vi "Test-FAMM.vi"() -> ()   [LabVIEW 2020]
doc: "Test the Historian performance"
uses:
  FAMM.lvclass
  HISW/HISW.lvclass
  <vilib>/platform/TimedLoop/XDataNode/XDataNode.xnode
  <vilib>/Platform/TimedLoop/XDataNode/nitl_modes.ctl
  <vilib>/Platform/TimedLoop/XDataNode/XDNodeRunTimeDep.lvlib
  <vilib>/Platform/TimedLoop/XDataNode/wakeup.ctl
  <vilib>/Platform/TimedLoop/XDataNode/timing_clust.ctl
  HISW/controls/typedef_PAQsample.ctl
  DBAL/DBAL.lvclass
  PAQ-memory.lvclass
panel:
  in  "View":bool
  in  "DAQ":bool
  out "# elements in queue":i32
  out "DAQ":picture
  in  "update":bool
  in  "auto":bool
  out "tablename":string
  out "Array":bool[](array[boolean])
  out "PAQpointers":i32[](array[numeric])
  out "XY Graph":cluster{"time":dbl[], "min":dbl[]}[](graph)
  in  "GET_Graph":bool
  in  "Size":i32=1000
  in  "Pointer":i32
  in  "TAG":i32=5 min=0 max=10000
  in  "Layer":i32 min=0
  out "Resolution":dbl format="%#.5p"
  out "Tags":i32
  out "Database configuration":string
  out "37x37":picture
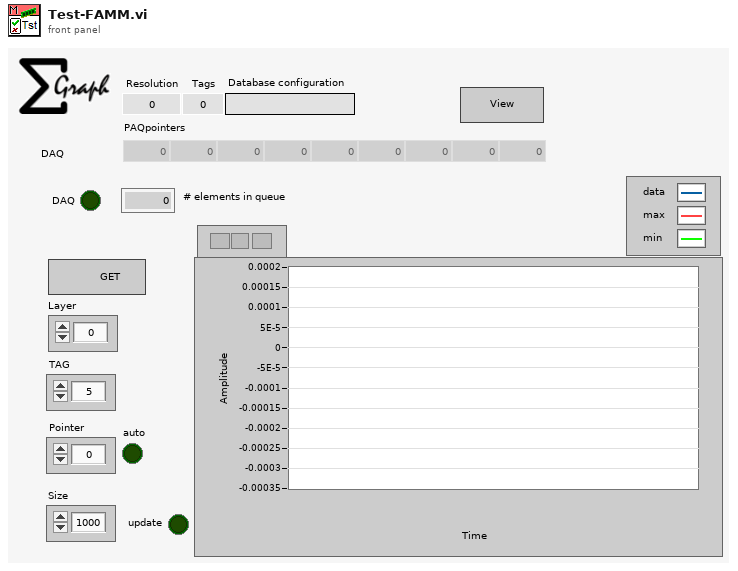
[diagram p1: front panel]
types:
  T1 = typedef "typedef_PAQsample.ctl" = cluster{"Time Stamp":timestamp, "TAGs":string[], "status":u32[], "data":dbl[], "Source":string}
  T2 = typedef "XDNodeRunTimeDep.lvlib/timing_clust.ctl" = cluster{"Expected End [f-1]":u64, "Actual End [f-1]":u64, "Finished Late? [f-1]":bool, "Expected End [i-1]":u64, "Actual End [i-1]":u64, "Finished Late? [i-1]":bool, "Expected Start [i]":u64, "Actual Start [i]":u64, "Expected Start [f]":u64, "Actual Start [f]":u64, "Source Name":string, "Structure Name":string, "Period":i64, "Deadline":i64, "Offset":i64, "Start":i64, "Priority":i32, "Timeout":i32, "Mode":T3, "Wakeup Reason":T4, "Error":errorcluster, "Source Type":string, "Secondary Source Type":string, "Global End Time":u64, "Global Start Time":u64, "Frame Duration":u64, "Iteration Duration":u64, "Assigned CPU":i32, "I/O Scan Engine Mode":u32}
  T3 = typedef "XDNodeRunTimeDep.lvlib/nitl_modes.ctl" = enum32{"No Change", "Process missed periods, maintain original phase", "Discard missed periods, maintain original phase", "Process missed periods, ignore original phase", "Discard missed periods, ignore original phase"}
  T4 = typedef "XDNodeRunTimeDep.lvlib/wakeup.ctl" = enum32{"Normal", "Aborted", "Asynchronous wakeup", "Timing source error", "Timed loop error", "Timeout"}
  T5 = cluster{"TAG":string, "Layer":i32, "Pointer":i32, "Size":i32}
  T6 = cluster{"time":dbl[], "data":dbl[], "max":dbl[], "min":dbl[], "status":u32[]}
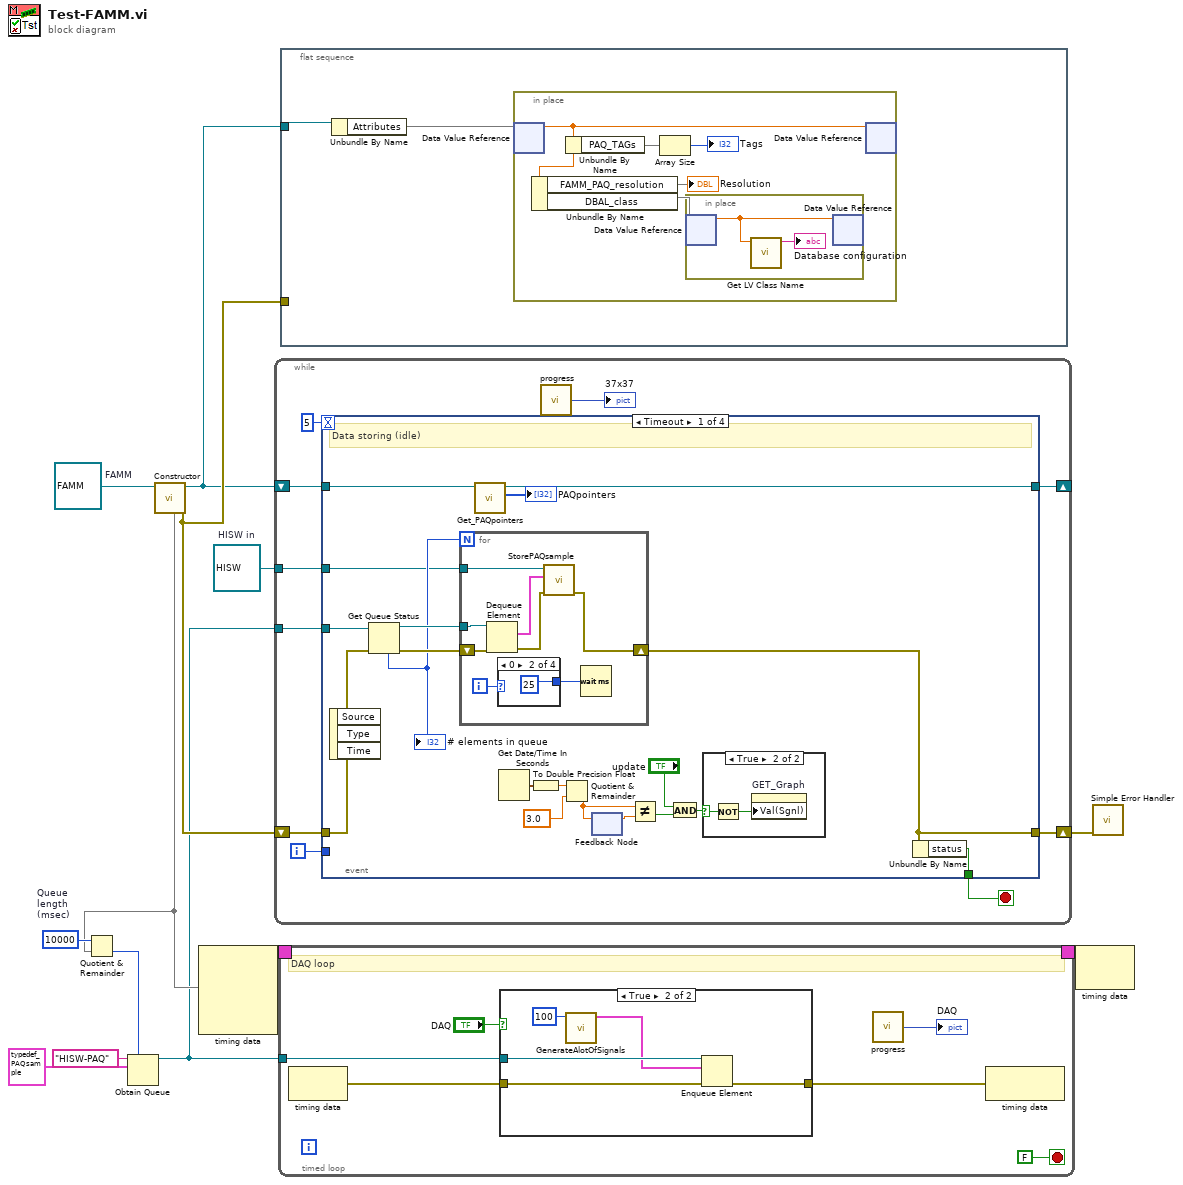
[diagram p0: block diagram]
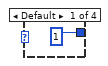
[diagram p3: hidden frame]
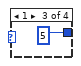
[diagram p4: hidden frame]
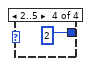
[diagram p5: hidden frame]
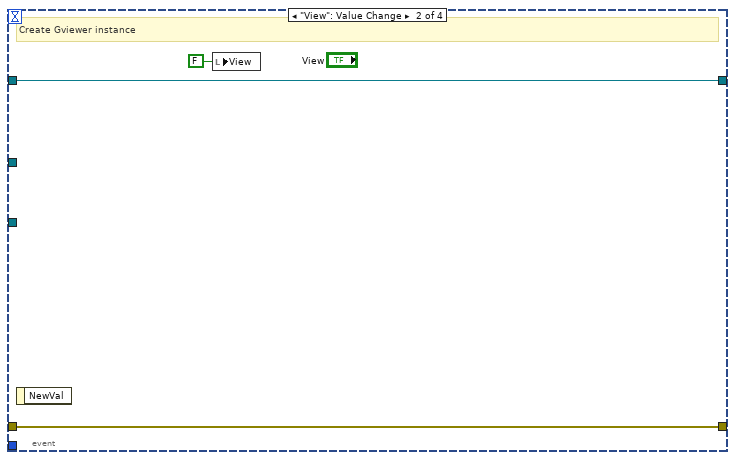
[diagram p7: hidden frame]
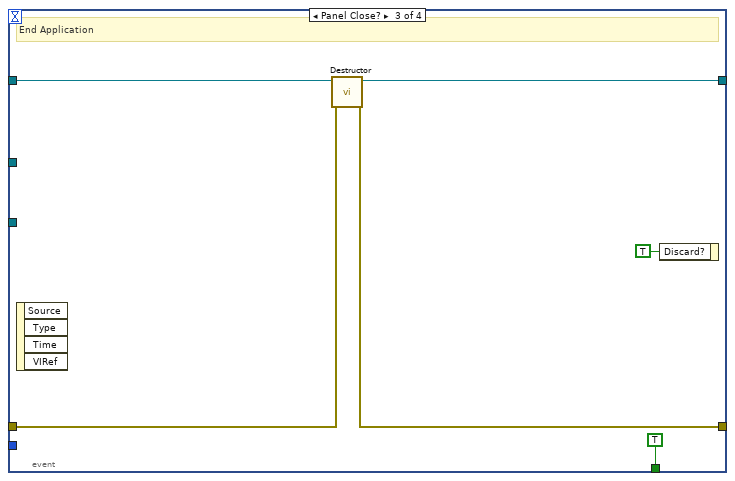
[diagram p8: hidden frame]
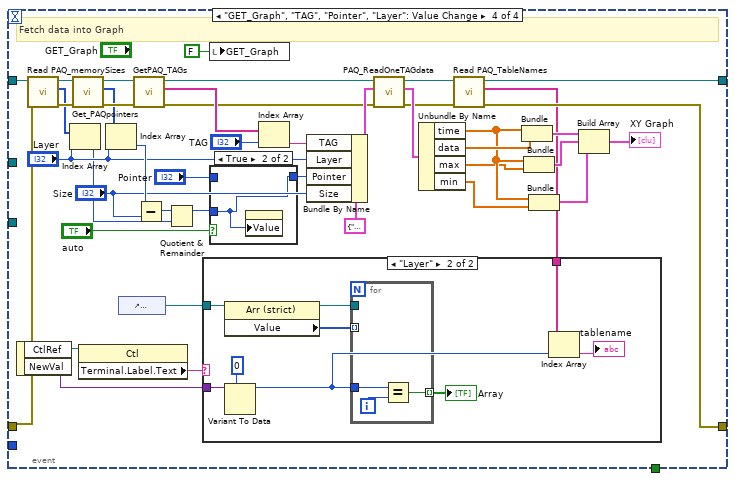
[diagram p9: hidden frame]
diagram:
  w5 = 10000  # Queue length (msec)
  w12 = refnum<class "HISW.lvclass"> refnum  # HISW in
  w13 = refnum<class "FAMM.lvclass"> refnum  # FAMM
  n1 = call "Constructor.vi"("FAMM in"=w13) -> ("error out"=w11:errorcluster, "FAMM out"=w1:refnum<class "FAMM.lvclass">, 4:w4)  [unwired: 6 in, 2 out]
  n2 = Quotient & Remainder(x=w5, y=w4) -> (floor(x/y)=w3:i32)  [unwired: 1 out]
  n3 = Obtain Queue(max queue size (-1, unlimited)=w3, name (unnamed)="HISW-PAQ", element data type=T1 {"Time Stamp"=timestamp(0 s since 1904-01-01), "TAGs"=[], "status"=[], "data"=[], "Source"=""} ("DAQ")) -> (queue out=w2:refnum<queue>)  [unwired: 2 in, 2 out]
  n4 = node-c288(w4) -> (w9:T2)  [unwired: 3 in]
  n5 = while {
    shift-right: [w22] -> _
    shift-left: w1 -> [w23]
    shift-right: [w18] -> w10
    shift-left: w11 -> [w20]
    tunnel: w12 -> [w21]
    tunnel: w2 -> [w14]
    i -> [w15]
    stop <- w19 stop-if-true
    n6 = event shown="[0] Timeout" {
      selector: _ -> [_ _ _ _]
      dyn-events: _ -> [_ _ _ _]
      timeout: 5 -> [_ _ _ _]
      tunnel: w23 -> [w41 w59 w63 w72]
      tunnel: [w40 w59 w62 w81] -> w22
      tunnel: w20 -> [w29 w58 w61 w68]
      tunnel: [w25 w58 w60 w79] -> w18
      tunnel: w21 -> [w24 _ _ _]
      tunnel: [w42 _ TRUE _] -> w19
      tunnel: w15 -> [_ _ _ _]
      tunnel: w14 -> [w30 _ _ _]
      event Timeout {
        # "Data storing (idle)"
        n7 = event-data() -> ()  [unwired: 1 in, 3 out]
        n8 = Get Queue Status(queue=w30, error in (no error)=w29) -> (queue out=w28:refnum<queue>, error out=w27:errorcluster, # elements in queue=w26:i32)  [unwired: 1 in, 5 out]
        "# elements in queue" <- w26
        n9 = for {
          N: w26 -> [_]
          tunnel: w28 -> [w50]
          shift-right: [w47] -> w25
          shift-left: w27 -> [w49]
          tunnel: w24 -> [w43]
          i -> [w45]
          n10 = Dequeue Element(queue=w50, error in (no error)=w49) -> (element=w46:T1, error out=w48:errorcluster)  [unwired: 1 in, 2 out]
          n11 = case shown="0" w45 {
            tunnel: [u32 1 ("milliseconds to wait") u32 25 ("milliseconds to wait") u32 5 ("milliseconds to wait") u32 2 ("milliseconds to wait")] -> w44
            frame Default {
            }
            frame 0 {
            }
            frame 1 {
            }
            frame 2..5 {
            }
          }
          n12 = call "StorePAQsample.vi"("error in (no error)"=w48, "PAQ IN"=w46, "HISW in"=w43) -> ("error out"=w47:errorcluster)  [unwired: 7 in, 1 out]
          n13 = Wait (ms)(milliseconds to wait=w44) -> ()  [unwired: 1 out]
        }
        n14 = call "Get_PAQpointers.vi"("FAMM in"=w41) -> ("PAQpointers"=→"PAQpointers":i32[], "FAMM out"=w40:refnum<class "FAMM.lvclass">)  [unwired: 8 in, 1 out]
        n15 = Get Date/Time In Seconds() -> (seconds since 1Jan1904=w38:timestamp)
        n16 = To Double Precision Float(number=w38) -> (double precision float=w37:dbl)
        n17 = Quotient & Remainder(x=w37, y=3.0) -> (floor(x/y)=w34:dbl)  [unwired: 1 out]
        n18 = feedback-in #1(w34) -> ()
        n19 = feedback #1() -> (w35:dbl)  [unwired: 1 in]
        n20 = Not Equal?(x=w34, y=w35) -> (x != y?=w33:bool)
        n21 = And(x="update", y=w33) -> (x .and. y?=w31:bool)
        n22 = case shown="True" w31 {
          selector: w31 -> [_ w56]
          frame False {
          }
          frame True {
            n23 = Not(x=w56) -> (.not. x?=w55:bool)
            n24 = property on="GET_Graph" class="Bool (strict)"("Val(Sgnl)"=w55) -> ()  [unwired: 2 in, 2 out]
          }
        }
        n25 = Unbundle By Name(w25) -> ("status"=w42:bool)
      }
      event "View": Value Change {
        # "Create Gviewer instance"
        n26 = event-data() -> ()  [unwired: 1 in, 1 out]
        n27 = local write "View"(FALSE ("View")) -> ()
      }
      event Panel Close? {
        # "End Application"
        n28 = event-data() -> ()  [unwired: 1 in, 4 out]
        n29 = call "Destructor.vi"("error in (no error)"=w61, "FAMM in"=w63) -> ("error out"=w60:errorcluster, "FAMM out"=w62:refnum<class "FAMM.lvclass">)  [unwired: 8 in]
        n30 = event-data("Discard?"=TRUE) -> ()  [unwired: 1 in, 1 out]
      }
      event "GET_Graph", "TAG", "Pointer", "Layer": Value Change {
        # "Fetch data into Graph"
        n31 = event-data() -> ("CtlRef"=w86:refnum<vi>, "NewVal"=w84:variant)  [unwired: 1 in]
        n32 = call "Read PAQ_memorySizes.vi"("error in (no error)"=w68, "FAMM in"=w72) -> ("error out"=w69:errorcluster, "Memory Size"=w67:i32[], "FAMM out"=w71:refnum<class "FAMM.lvclass">)  [unwired: 7 in]
        n33 = Index Array(array=w67, index="Layer") -> (element=w66:i32)
        n34 = call "Get_PAQpointers.vi"("error in (no error)"=w69, "FAMM in"=w71) -> ("error out"=w90:errorcluster, "PAQpointers"=w89:i32[], "FAMM out"=w91:refnum<class "FAMM.lvclass">)  [unwired: 7 in]
        n35 = property class="Ctl"(reference=w86) -> ("Terminal.Label.Text"=w85:string)  [unwired: 1 in, 2 out]
        n36 = Index Array(array=w89, index="Layer") -> (element=w88:i32)
        n37 = control-ref of="PAQpointers"() -> (w83:refnum<vi>)
        n38 = call "GetPAQ_TAGs.vi"("error in (no error)"=w90, "FAMM in"=w91) -> ("error out"=w101:errorcluster, "PAQ_TAGs"=w102:string[], "FAMM out"=w100:refnum<class "FAMM.lvclass">)  [unwired: 7 in]
        n39 = Subtract(x=w88, y="Size") -> (x-y=w74:i32)
        n40 = Quotient & Remainder(x=w74, y=w66) -> (x-y*floor(x/y)=w73:i32)  [unwired: 1 out]
        n41 = local write "GET_Graph"(FALSE ("GET_Graph")) -> ()
        n42 = case shown="True" "auto" {
          tunnel: w73 -> [_ w110]
          tunnel: [w109 w110] -> w76
          tunnel: "Pointer" -> [w109 _]
          frame False {
          }
          frame True {
            n43 = property on="Pointer" class="DigNum (strict)"("Value"=w110) -> ()  [unwired: 2 in, 2 out]
          }
        }
        n44 = Index Array(array=w102, index="TAG") -> (element=w103:string)
        n45 = Bundle By Name(cluster=T5 {"TAG"="", "Layer"=0, "Pointer"=0, "Size"=1000} ("FetchInfo"), "TAG"=w103, "Layer"="Layer", "Pointer"=w76, "Size"="Size") -> (w104:T5)
        n46 = call "PAQ_ReadOneTAGdata.vi"("error in (no error)"=w101, "FetchInfo"=w104, "FAMM in"=w100) -> ("error out"=w80:errorcluster, "GraphData"=w106:T6, "FAMM out"=w82:refnum<class "FAMM.lvclass">)  [unwired: 6 in]
        n47 = Unbundle By Name(w106) -> ("time"=w98:dbl[], "data"=w99:dbl[], "max"=w97:dbl[], "min"=w96:dbl[])
        n48 = call "Read PAQ_TableNames.vi"("error in (no error)"=w80, "FAMM in"=w82) -> ("error out"=w79:errorcluster, "TableNames"=w78:string[], "FAMM out"=w81:refnum<class "FAMM.lvclass">)  [unwired: 7 in]
        n49 = case shown="\"Layer\"" w85 {
          tunnel: w84 -> [_ w119]
          tunnel: w83 -> [_ w117]
          tunnel: w78 -> [_ w111]
          frame Default {
          }
          frame "Layer" {
            n50 = property class="Arr (strict)"(reference=w117) -> (reference out=w115:refnum<vi>, "Value"=w116:i32[])  [unwired: 1 in, 1 out]
            n51 = Variant To Data(type=0 ("Layer"), Variant=w119) -> (data=w113:i32)  [unwired: 1 in, 1 out]
            n52 = for {
              tunnel: w116 -> [_] mode=indexing
              tunnel: w115 -> [_]
              tunnel: w113 -> [w122]
              tunnel: [w120] -> w114 mode=indexing
              i -> [w121]
              n53 = Equal?(x=w122, y=w121) -> (x = y?=w120:bool)
            }
            "Array" <- w114
            n54 = Index Array(array=w111, index=w113) -> (element=→"tablename":string)
          }
        }
        n55 = Bundle("time"=w98, "data"=w99) -> (w95:cluster{"time":dbl[], "data":dbl[]})  [unwired: 1 in]
        n56 = Bundle("time"=w98, "max"=w97) -> (w94:cluster{"time":dbl[], "max":dbl[]})  [unwired: 1 in]
        n57 = Bundle("time"=w98, "min"=w96) -> (w93:cluster{"time":dbl[], "min":dbl[]})  [unwired: 1 in]
        n58 = Build Array(w95, w94, w93) -> (→"XY Graph":cluster{"time":dbl[], "min":dbl[]}[])
      }
    }
    n59 = call "progress.vi"() -> ("37x37"=→"37x37":picture)  [unwired: 7 in]
  }
  n60 = timed-loop {
    timing: w9 -> [_]
    timing-out: [_] -> w8
    tunnel: w2 -> [w126]
    stop <- FALSE stop-if-true
    # "DAQ loop"
    n61 = node-c288() -> (w125:errorcluster)  [unwired: 1 in]
    n62 = case shown="True" "DAQ" {
      tunnel: w126 -> [_ w134]
      tunnel: w125 -> [w129 w133]
      tunnel: [w129 w132] -> w124
      frame False {
      }
      frame True {
        n63 = call "GenerateAlotOfSignals.vi"("Channels"=100) -> ("DAQ"=w130:T1)  [unwired: 10 in]
        n64 = Enqueue Element(queue=w134, element=w130, error in (no error)=w133) -> (error out=w132:errorcluster)  [unwired: 1 in, 2 out]
      }
    }
    n65 = call "progress.vi"() -> ("37x37"=→"DAQ":picture)  [unwired: 7 in]
    n66 = node-c288(w124) -> ()  [unwired: 1 out]
  }
  n67 = flat-sequence {
    tunnel: w11 -> [_]
    tunnel: w1 -> [w141]
    frame #0 {
      n68 = Unbundle By Name(w141) -> ("Attributes"=w140)
      n69 = in-place {
        n70 = in-place-dvr #2(w140) -> (w142:dbl)  [unwired: 1 out]
        n71 = Unbundle By Name(w142) -> ("FAMM_PAQ_resolution"=→"Resolution", "DBAL_class"=w144)
        n72 = Unbundle By Name(w142) -> ("PAQ_TAGs"=w146)
        n73 = Array Size(array=w146) -> (size(s)=→"Tags":i32)
        n74 = in-place {
          n75 = in-place-dvr #3(w144) -> (w148:dbl)  [unwired: 1 out]
          n76 = call <vilib>:"Get LV Class Name.vi"("object"=w148) -> ("class name"=→"Database configuration":string)  [unwired: 9 in, 1 out]
          n77 = in-place-dvr #3(w148) -> ()  [unwired: 2 out]
        }
        n78 = in-place-dvr #2(w142) -> ()  [unwired: 2 out]
      }
    }
  }
  n79 = node-c288(w8) -> ()  [unwired: 1 out]
  n80 = call <vilib>:"Simple Error Handler.vi"("error in (no error)"=w10) -> ()  [unwired: 4 in, 5 out]
